vi "RemoteVI Send Window Frame.vi"(0 "Client":T1, 1 "height":i32, 2 "last sent":u32[][](array[numeric]), 5 "id":u64, 7 "pixmap":u32[][](array[numeric]), 9 "width":i32, 11 "error in":errorcluster) -> (4 "Client out":T1, 6 "last sent out":u32[][](array[numeric]), 8 "sent?":bool, 15 "error out":errorcluster)   [LabVIEW 2020, in "RemoteVI.lvlib"]
doc: "Sends one WINDOW FRAME of one listed window to one client if flow control allows (docs\\protocol.md sections 5 and 7) - RemoteVI Send Frame.vi for another window. Nothing happens when the client is closed or already has 2 unacknowledged frames (seq - acked >= 2, the seq is shared with FRAME), when the capture is empty (the window could not be drawn), or when RemoteVI Dirty Rects.vi finds no change against last sent - the picture of THIS window this client was last sent; an empty last sent (a window the client has not seen yet) or a size change gives the whole window. Otherwise every dirty rect is encoded with RemoteVI Encode Rect PNG.vi, the message is built with RemoteVI Window Frame Encode.vi (id, seq + 1, width, height), wrapped in a binary WebSocket frame and written with TCP Write (2 s timeout). On success seq is incremented, last sent out becomes pixmap and sent? is TRUE; a write error sets closed instead. error out carries PNG encoding errors."
uses:
  RemoteVI.lvlib
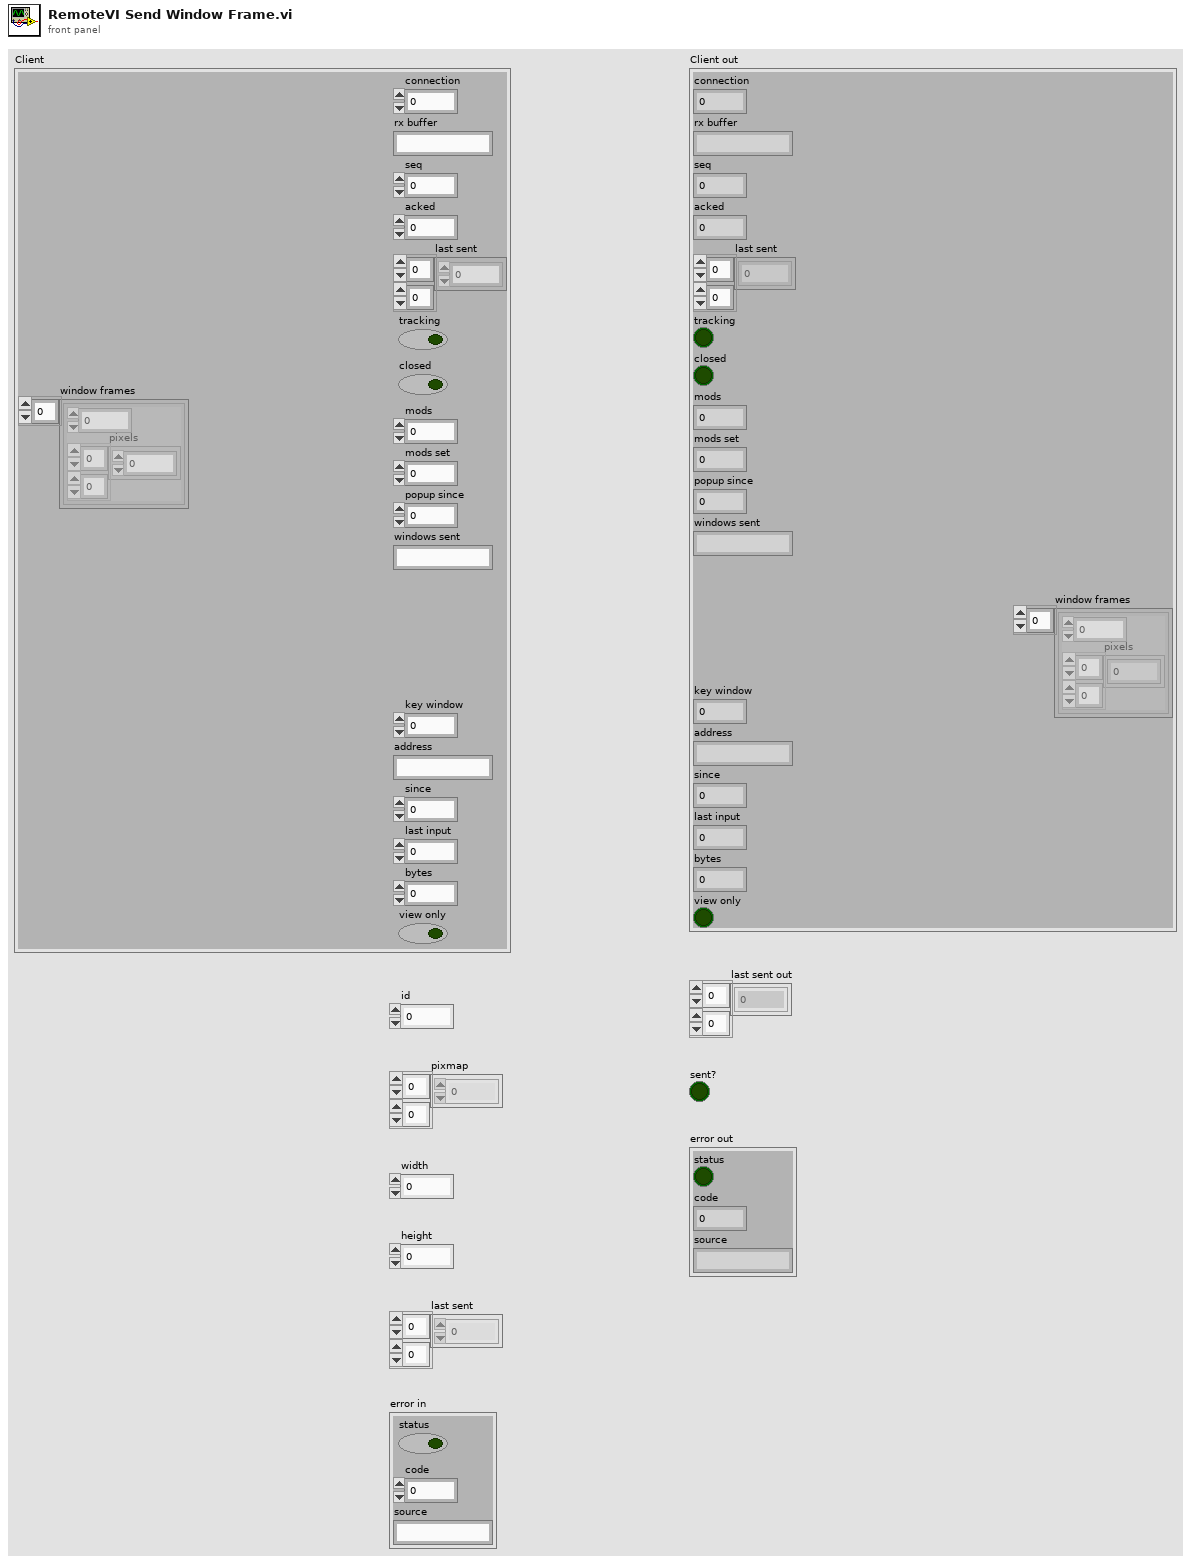
[diagram p1: front panel]
types:
  T1 = cluster{"connection":u32, "rx buffer":string, "seq":u32, "acked":u32, "last sent":u32[][], "tracking":bool, "closed":bool, "mods":u8, "mods set":u8, "popup since":u32, "windows sent":string, "window frames":cluster{"id":u64, "pixels":u32[][]}[], "key window":u64, "address":string, "since":dbl, "last input":dbl, "bytes":dbl, "view only":bool}
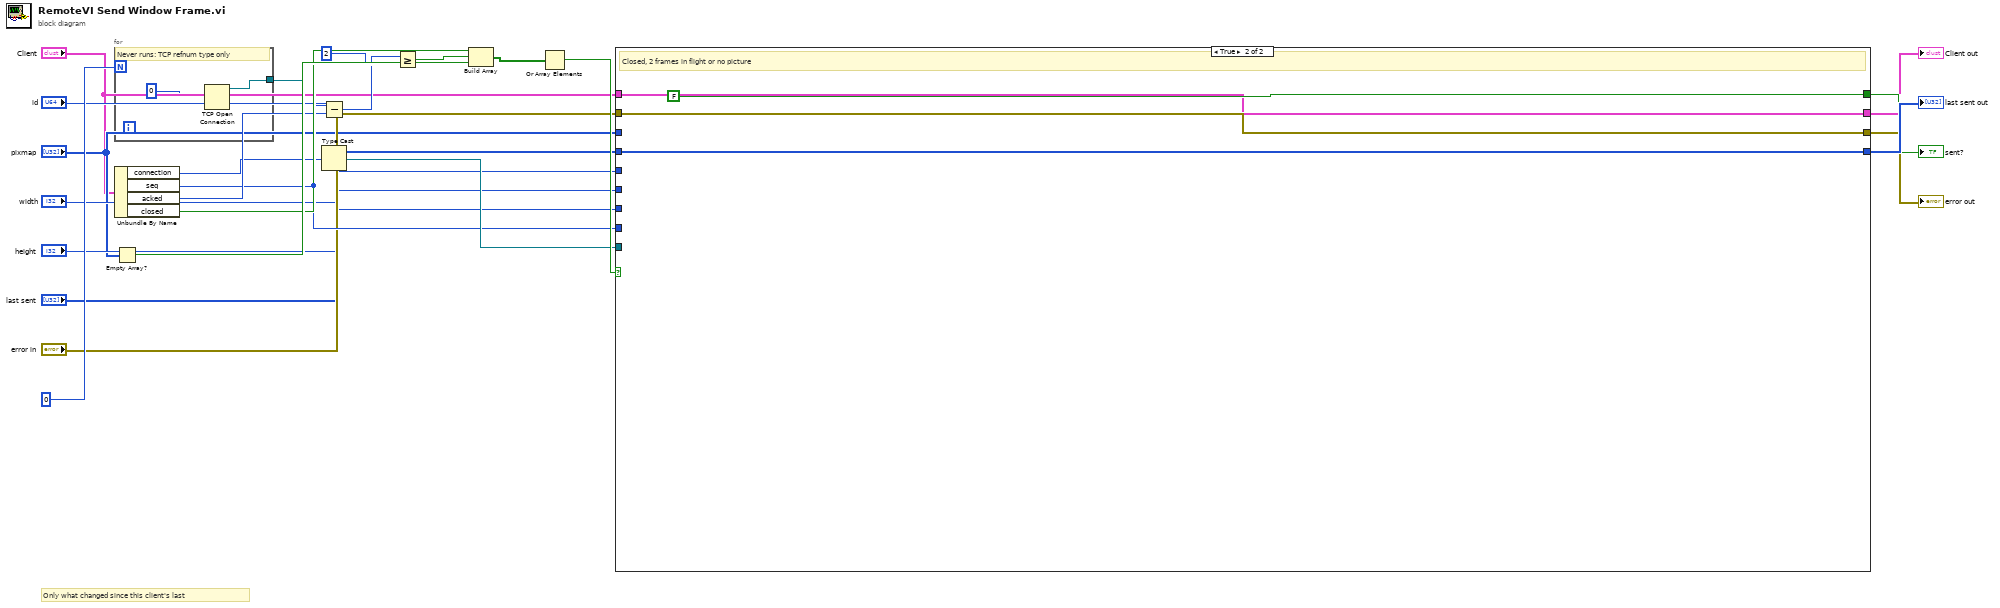
[diagram p0: block diagram]
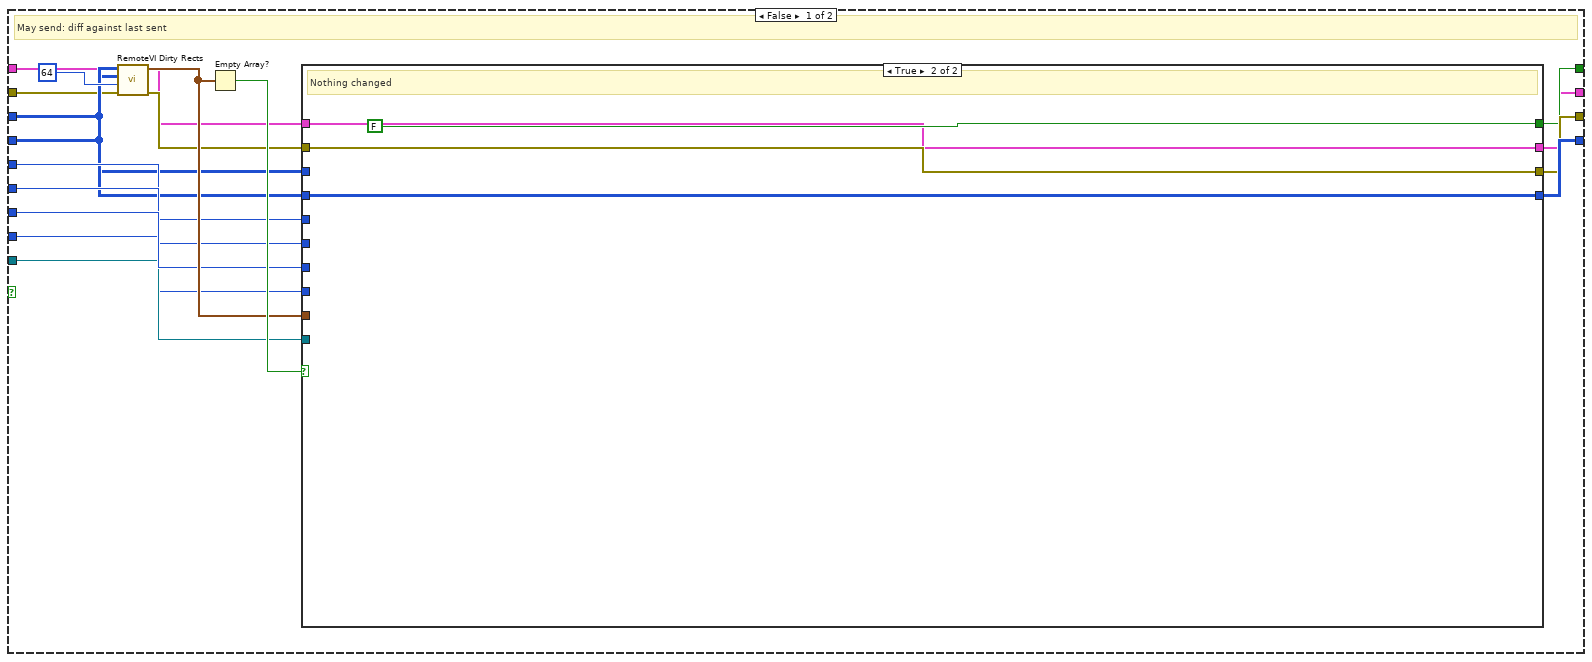
[diagram p2: hidden frame]
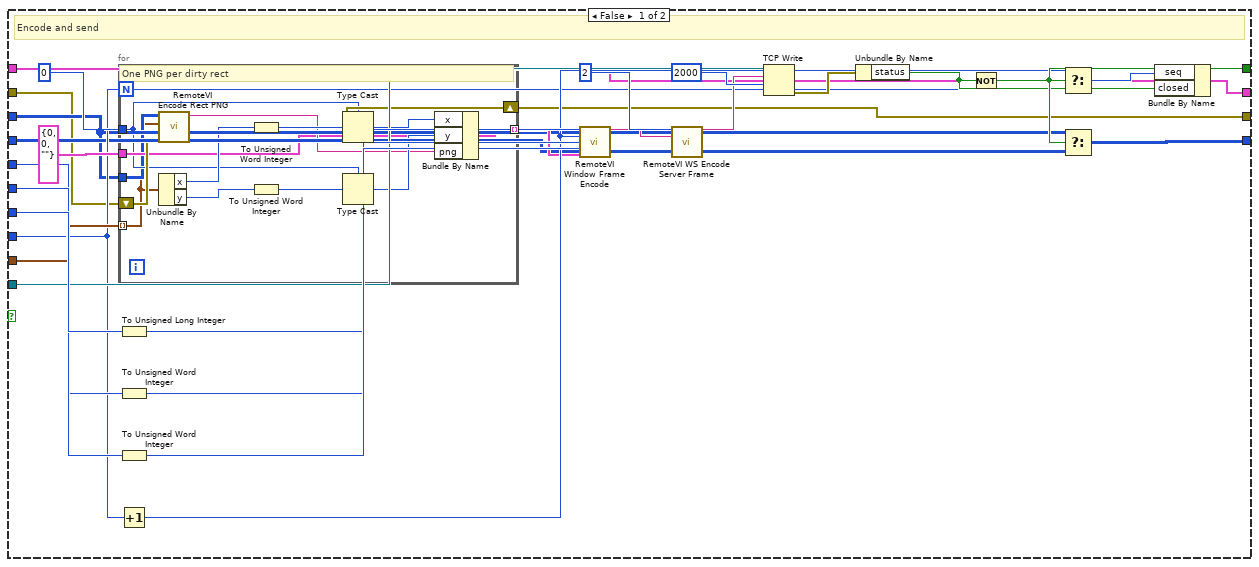
[diagram p3: hidden frame]
diagram:
  # "Only what changed since this client's last"
  n1 = for {
    N: 0 -> [_]
    tunnel: [w26] -> w9
    # "Never runs: TCP refnum type only"
    n2 = TCP Open Connection(remote port or service name=u16 0) -> (connection ID=w26:refnum<k5>)  [unwired: 4 in, 1 out]
  }
  n3 = Unbundle By Name("Client") -> ("connection"=w10:u32, "seq"=w11:u32, "acked"=w12:u32, "closed"=w13:bool)
  n4 = Empty Array?(array="pixmap") -> (empty?=w18:bool)
  n5 = Subtract(x=w11, y=w12) -> (x-y=w15:u32)
  n6 = Type Cast(type=w9, x=w10) -> (*(type *) &x=w14:refnum<k5>)
  n7 = Greater Or Equal?(x=w15, y=u32 2) -> (x >= y?=w17:bool)
  n8 = Build Array(w13, w17, w18) -> (w19:bool[])
  n9 = Or Array Elements(Boolean array=w19) -> (logical OR=w20:bool)
  n10 = case shown="True" w20 {
    tunnel: "Client" -> [w27 w89]
    tunnel: "error in" -> [w28 w90]
    tunnel: "pixmap" -> [w29 _]
    tunnel: "last sent" -> [w30 w91]
    tunnel: "width" -> [w33 _]
    tunnel: "height" -> [w34 _]
    tunnel: "id" -> [w35 _]
    tunnel: [w40 FALSE] -> w22
    tunnel: w11 -> [w31 _]
    tunnel: [w39 w89] -> w21
    tunnel: [w41 w90] -> w23
    tunnel: [w42 w91] -> w24
    tunnel: w14 -> [w32 _]
    frame False {
      # "May send: diff against last sent"
      n11 = call "RemoteVI Dirty Rects.vi"("tile size"=64, "current"=w29, "previous"=w30) -> ("rects"=w37:cluster{"x":i32, "y":i32, "w":i32, "h":i32}[])  [unwired: 8 in]
      n12 = Empty Array?(array=w37) -> (empty?=w38:bool)
      n13 = case shown="True" w38 {
        tunnel: [w67 FALSE] -> w40
        tunnel: w27 -> [w43 w85]
        tunnel: w28 -> [w44 w86]
        tunnel: w29 -> [w45 _]
        tunnel: w30 -> [w46 w87]
        tunnel: w33 -> [w49 _]
        tunnel: w34 -> [w50 _]
        tunnel: w35 -> [w52 _]
        tunnel: w31 -> [w47 _]
        tunnel: w37 -> [w51 _]
        tunnel: [w70 w85] -> w39
        tunnel: [w55 w86] -> w41
        tunnel: [w69 w87] -> w42
        tunnel: w32 -> [w48 _]
        frame False {
          # "Encode and send"
          n14 = for {
            tunnel: i16 0 -> [w73]
            tunnel: cluster{"x":i16, "y":i16, "png":string} {"x"=0, "y"=0, "png"=""} -> [w74]
            tunnel: w45 -> [w72]
            shift-right: [w76] -> w55
            shift-left: w44 -> [w75]
            tunnel: w51 -> [w71] mode=indexing
            tunnel: [w84] -> w56 mode=indexing
            # "One PNG per dirty rect"
            n15 = call "RemoteVI Encode Rect PNG.vi"("error in"=w75, "rect"=w71, "pixmap"=w72) -> ("error out"=w76:errorcluster, "png"=w77:string)  [unwired: 7 in]
            n16 = Unbundle By Name(w71) -> ("x"=w78:i32, "y"=w79:i32)
            n17 = To Unsigned Word Integer(number=w78) -> (unsigned 16bit integer=w80:u16)
            n18 = To Unsigned Word Integer(number=w79) -> (unsigned 16bit integer=w81:u16)
            n19 = Type Cast(type=w73, x=w80) -> (*(type *) &x=w82:i16)
            n20 = Type Cast(type=w73, x=w81) -> (*(type *) &x=w83:i16)
            n21 = Bundle By Name(cluster=w74, "x"=w82, "y"=w83, "png"=w77) -> (w84:cluster{"x":i16, "y":i16, "png":string})
          }
          n22 = To Unsigned Long Integer(number=w52) -> (unsigned 32bit integer=w58:u32)
          n23 = To Unsigned Word Integer(number=w49) -> (unsigned 16bit integer=w59:u16)
          n24 = To Unsigned Word Integer(number=w50) -> (unsigned 16bit integer=w60:u16)
          n25 = Increment(x=w47) -> (x+1=w57:u32)
          n26 = call "RemoteVI Window Frame Encode.vi"("id"=w58, "seq"=w57, "width"=w59, "height"=w60, "rects"=w56) -> ("message"=w61:string)  [unwired: 10 in]
          n27 = call "RemoteVI WS Encode Server Frame.vi"("opcode"=u8 2, "payload"=w61) -> ("frame"=w63:string)  [unwired: 13 in]
          n28 = TCP Write(connection ID=w48, data in=w63, 9:2000) -> (error out=w65:errorcluster)  [unwired: 1 in, 2 out]
          n29 = Unbundle By Name(w65) -> ("status"=w66:bool)
          n30 = Not(x=w66) -> (.not. x?=w67:bool)
          n31 = Select(t=w57, s=w67, f=w47) -> (s? t:f=w68:u32)
          n32 = Select(t=w45, s=w67, f=w46) -> (s? t:f=w69:u32[][])
          n33 = Bundle By Name(cluster=w43, "seq"=w68, "closed"=w66) -> (w70:T1)
        }
        frame True {
          # "Nothing changed"
        }
      }
    }
    frame True {
      # "Closed, 2 frames in flight or no picture"
    }
  }
  "Client out" <- w21
  "last sent out" <- w24
  "sent?" <- w22
  "error out" <- w23
